vi "subFirmware.vi"(1 "Index":i32=1) -> ()   [LabVIEW 2020]
panel:
  in  "Reset drives":bool
  in  "Reset board":bool
  out "Interface":string
  out "Sernum":string caption="Serial number"
  in  "Close":bool
  out "Version":string caption="Board firmware"
  # "Control unit"
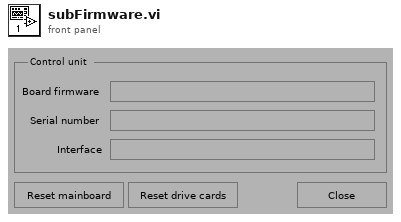
[diagram p1: front panel]
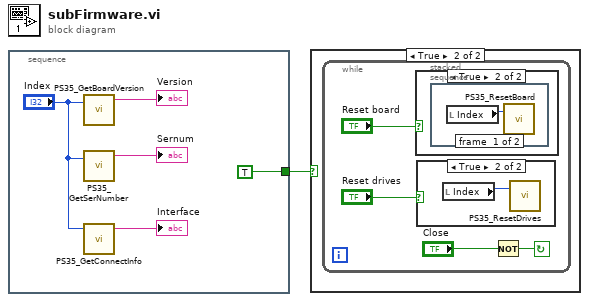
[diagram p0: block diagram]
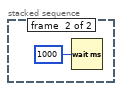
[diagram p5: hidden frame]
diagram:
  n1 = stacked-sequence {
    tunnel: [TRUE] -> w1
    frame #0 {
      n2 = call "PS35_GetBoardVersion.vi"("Control unit ID"="Index") -> ("Board version"=→"Version":string)  [unwired: 1 in, 2 out]
      n3 = call "PS35_GetSerNumber.vi"("Control unit ID"="Index") -> ("Serial number"=→"Sernum":string)  [unwired: 1 in, 2 out]
      n4 = call "PS35_GetConnectInfo.vi"("Control unit ID"="Index") -> ("Connecting info"=→"Interface":string)  [unwired: 2 in, 2 out]
    }
  }
  n5 = case shown="True" w1 {
    frame False {
    }
    frame True {
      n6 = while {
        stop <- w10 continue-if-true
        n7 = case shown="True" "Reset board" {
          frame False {
          }
          frame True {
            n8 = stacked-sequence {
              frame #0 {
                n9 = local read "Index"() -> (w12:i32)
                n10 = call "PS35_ResetBoard.vi"("Control unit ID"=w12) -> ()  [unwired: 2 in, 1 out]
              }
              frame #1 {
                n11 = Wait (ms)(milliseconds to wait=u32 1000) -> ()  [unwired: 1 out]
              }
            }
          }
        }
        n12 = case shown="True" "Reset drives" {
          frame False {
          }
          frame True {
            n13 = local read "Index"() -> (w11:i32)
            n14 = call "PS35_ResetDrives.vi"("Control unit ID"=w11) -> ()  [unwired: 2 in, 1 out]
          }
        }
        n15 = Not(x="Close") -> (.not. x?=w10:bool)
      }
    }
  }
